vi "CaptureWave.vi"(0 "UCI_DllPath":path, 1 "Command":string(combo)="capture wave:.bin@CH:0@DT:vol;", 5 "Session_id":i32, 7 "Length":u32, 9 "InputData":u8[](array[numeric]), 11 "Timeout(ms)":u32, 12 "ReadType":enum16{"bin", "csv"}(ring)) -> (4 "OutputData":sgl[](array[numeric]), 10 "ResultDescription":string, 15 ".csv File Path":string)   [LabVIEW 2015]
panel:
  out "ReadOutputData":u8[](array[numeric]) format="%02x"
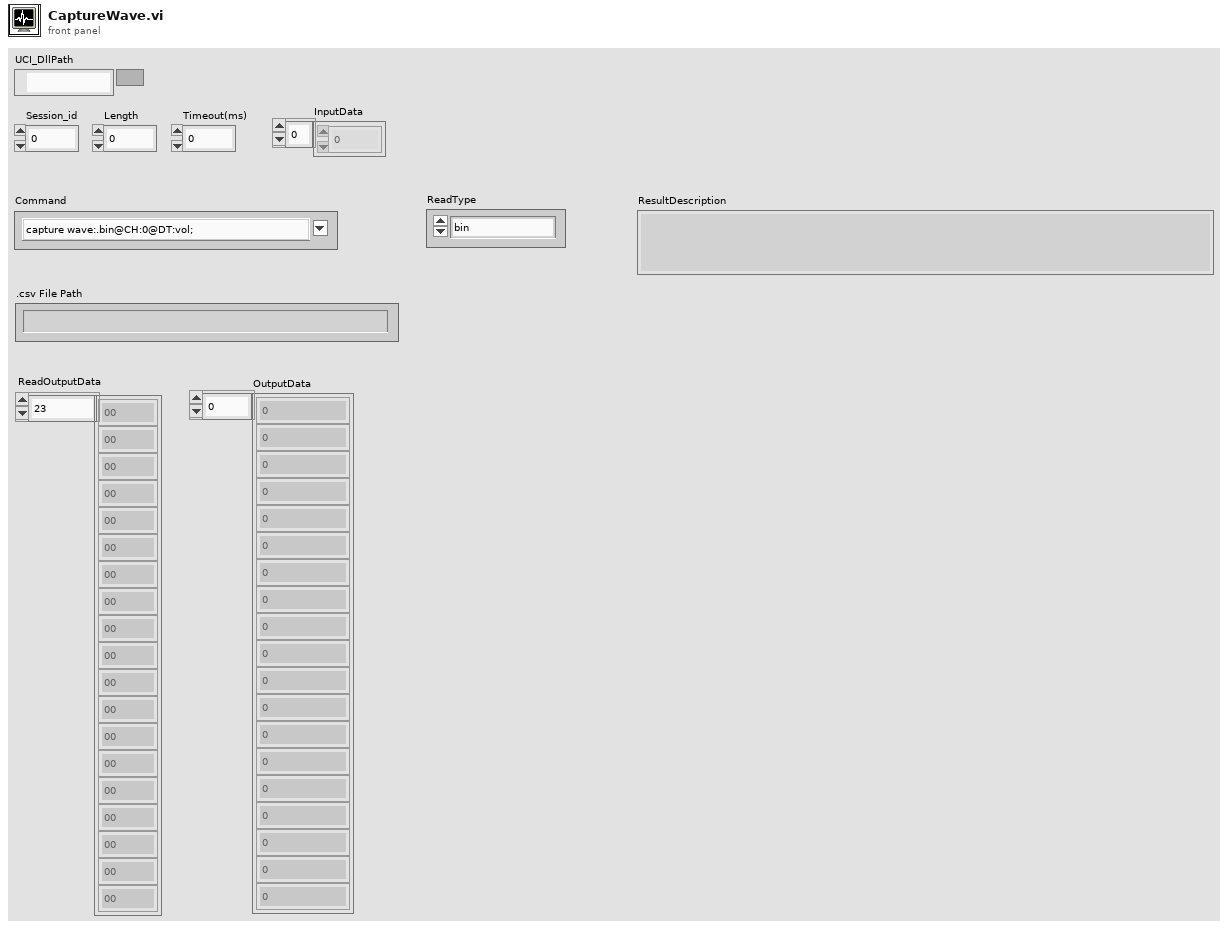
[diagram p1: front panel]
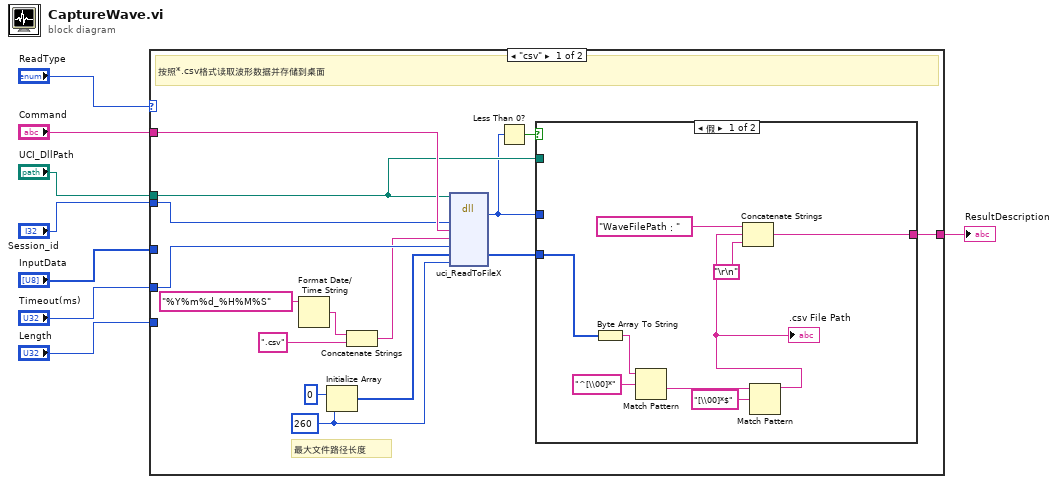
[diagram p0: block diagram]
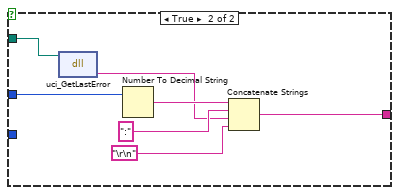
[diagram p2: hidden frame]
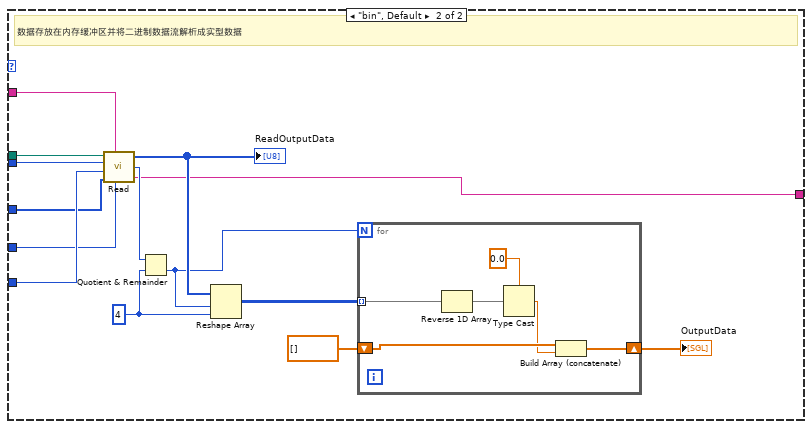
[diagram p3: hidden frame]
diagram:
  n1 = case shown="\"csv\"" "ReadType" {
    tunnel: "Session_id" -> [w22 w51]
    tunnel: "Length" -> [_ w50]
    tunnel: "Command" -> [w23 w53]
    tunnel: "UCI_DllPath" -> [w12 w52]
    tunnel: "Timeout(ms)" -> [w21 w42]
    tunnel: [w11 w41] -> w2
    tunnel: "InputData" -> [_ w40]
    frame "csv" {
      w17 = 260 ("维数大小")
      # "最大文件路径长度"
      # "按照*.csv格式读取波形数据并存储到桌面"
      n2 = Format Date/Time String(time format string (%c)="%Y%m%d_%H%M%S" ("时间格式字符串(%c)")) -> (date/time string=w15:string)  [unwired: 2 in]
      n3 = Initialize Array(u8 0 ("元素"), w17) -> (w19:u8[])
      n4 = Concatenate Strings(w15, ".csv" ("_filePath")) -> (w13:string)
      n5 = dll-call lib="E:/JL-Project/LabView-Project/ASCII/uci.dll" fn="uci_ReadToFileX"(path in=w12, "_session"=w22, "_msg"=w23, "_filePath"=w13, "_timeout"=w21, "_filePathFinal"=w19, "_filePathFinalLength"=w17) -> ("返回类型"=w10:i32, "_filePathFinal"=w18:u8[])  [unwired: 7 in, 2 out]
      n6 = Less Than 0?(x=w10) -> (x < 0?=w9:bool)
      n7 = case shown="假" w9 {
        tunnel: w18 -> [w32 _]
        tunnel: w12 -> [_ w39]
        tunnel: w10 -> [_ w35]
        tunnel: [w30 w34] -> w11
        frame False {
          n8 = Byte Array To String(unsigned byte array=w32) -> (string=w25:string)
          n9 = Match Pattern(string=w25, regular expression="^[\\00]*") -> (after substring=w28:string)  [unwired: 1 in, 3 out]
          n10 = Match Pattern(string=w28, regular expression="[\\00]*$") -> (before substring=w24:string)  [unwired: 1 in, 3 out]
          ".csv File Path" <- w24
          n11 = Concatenate Strings("WaveFilePath：" ("字符串"), w24, "\r\n") -> (w30:string)
        }
        frame True {
          n12 = dll-call lib="E:/JL-Project/LabView-Project/ASCII/uci.dll" fn="uci_GetLastError"(path in=w39) -> ("返回类型"=w36:string)  [unwired: 2 in, 2 out]
          n13 = Number To Decimal String(number=w35) -> (decimal integer string=w38:string)  [unwired: 1 in]
          n14 = Concatenate Strings(w38, ":" ("字符串"), w36, "\r\n") -> (w34:string)
        }
      }
    }
    frame "bin", Default {
      w47 = 4 ("维数大小")
      # "数据存放在内存缓冲区并将二进制数据流解析成实型数据"
      n15 = call "Read.vi"("UCI_DllPath"=w52, "Command"=w53, "Session_id"=w51, "Length"=w50, "Timeout"=w42, "InputData"=w40) -> ("OutputData"=w49:u8[], "Result"=w48:i32, "ResultDescription"=w41:string)
      "ReadOutputData" <- w49
      n16 = Quotient & Remainder(x=w48, y=w47) -> (floor(x/y)=w46:i32)  [unwired: 1 out]
      n17 = Reshape Array(w49, w46, w47) -> (w45:u8[][])
      n18 = for {
        N: w46 -> [_]
        tunnel: w45 -> [w57] mode=indexing
        shift-right: [w56] -> w43
        shift-left: sgl[] [] -> [w55]
        n19 = Reverse 1D Array(array=w57) -> (reversed array=w58:u8[])
        n20 = Type Cast(type=sgl 0.0 ("类型"), x=w58) -> (*(type *) &x=w54:sgl)
        n21 = Build Array (concatenate)(w55, w54) -> (w56:sgl[])
      }
      "OutputData" <- w43
    }
  }
  "ResultDescription" <- w2
